vi "Latest.vi"(8 "error in (no error)":errorcluster, 10 "Migrations Folder":path, 11 "SQLite Connection in":refnum<class "Connection.lvclass">) -> (0 "error out":errorcluster, 3 "SQLite Connection out":refnum<class "Connection.lvclass">)   [LabVIEW 2024, in "DBMigrations.lvlib"]
doc: "Update database to latest version."
uses:
  DBMigrations.lvlib
  <vilib>/drjdpowell/SQLite Library/SQL Connection/Connection.lvclass
  4642a8a4-5c78-40db-aa34-a8ecced09657.vi
  <vilib>/drjdpowell/SQLite Library/SQL Connection/Execute SQL (Single Integer).vi
  <vilib>/Comparison/Less/Less Functor/Less Functor.lvclass
  <vilib>/drjdpowell/SQLite Library/SQLite.lvlib
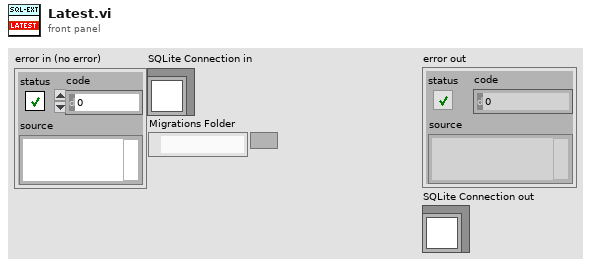
[diagram p1: front panel]
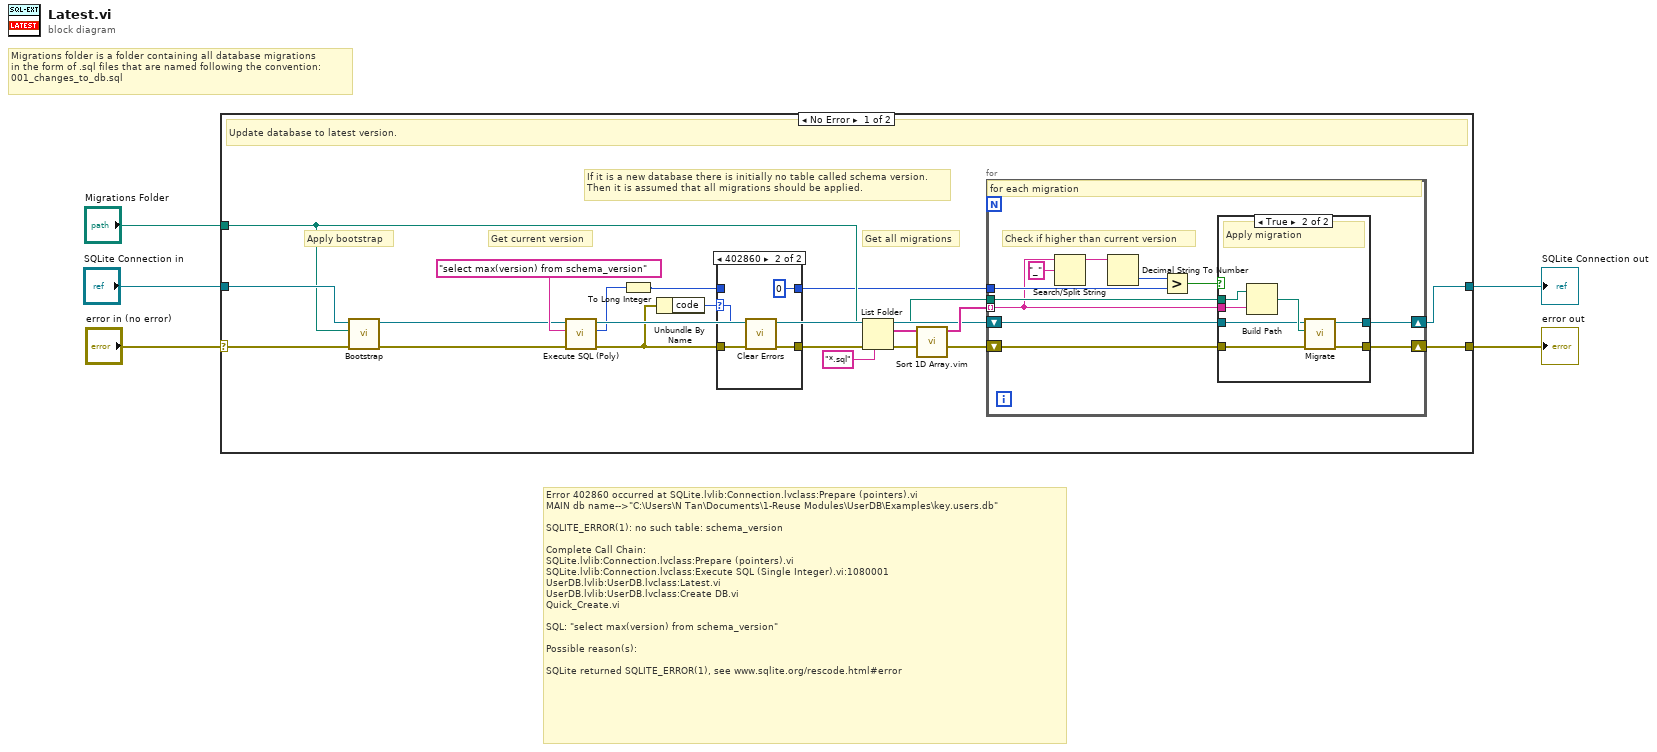
[diagram p0: block diagram]
diagram:
  # "Error 402860 occurred at SQLite.lvlib:Connection.lvclass:Prepare (pointers).vi\nMAIN db name-->\"C:\\Users\\N Tan\\Documents\\1-Reuse Modules\\UserDB\\Examples\\key.users.db\"\n\nSQLITE_ERROR(1): no such table: schema_version\n\nComplete Call Chain:\nSQLite.lvlib:Connection.lvclass:Prepare (pointers).vi\nSQLite.lvlib:Connection.lvclass:Execute SQL (Single Integer).vi:1080001\nUserDB.lvlib:UserDB.lvclass:Latest.vi\nUserDB.lvlib:UserDB.lvclass:Create DB.vi\nQuick_Create.vi\n\nSQL: \"select max(version) from schema_version\"\n\nPossible reason(s):\n\nSQLite returned SQLITE_ERROR(1), see www.sqlite.org/rescode.html#error"
  # "Migrations folder is a folder containing all database migrations\nin the form of .sql files that are named following the convention:\n001_changes_to_db.sql"
  n1 = case shown="No Error" "error in (no error)" {
    selector: "error in (no error)" -> [w15 w53]
    tunnel: [w21 w53] -> w5
    tunnel: "SQLite Connection in" -> [w14 w52]
    tunnel: [w18 w52] -> w2
    tunnel: "Migrations Folder" -> [w13 _]
    frame No Error {
      # "If it is a new database there is initially no table called schema version.\nThen it is assumed that all migrations should be applied."
      # "Get current version"
      # "Apply bootstrap"
      # "Get all migrations"
      # "Update database to latest version."
      n2 = call "Bootstrap.vi"("error in (no error)"=w15, "Migrations Folder"=w13, "SQLite Connection in"=w14) -> ("error out"=w12:errorcluster, "SQLite Connection out"=w11:refnum<class "Connection.lvclass">)  [unwired: 7 in]
      n3 = call-poly <vilib>:"Execute SQL (Poly).vi"("error in (no error)"=w12, "SQL"="select max(version) from schema_version", "SQLite Connection in"=w11) -> ("error out"=w9:errorcluster, "Result"=w16:i64, "SQLite Connection"=w20:refnum<class "Connection.lvclass">)  [unwired: 6 in]
      n4 = To Long Integer(number=w16) -> (32bit integer=w8:i32)
      n5 = Unbundle By Name(w9) -> ("code"=w10:i32)
      n6 = case shown="402860" w10 {
        selector: w10 -> [_ w28]
        tunnel: w9 -> [w27 w30]
        tunnel: [w27 w29] -> w7
        tunnel: w8 -> [w26 _]
        tunnel: [w26 0] -> w6
        frame 0, Default {
        }
        frame 402860 {
          n7 = call <vilib>:"Clear Errors.vi"("error in (no error)"=w30, "specific error code to clear (0: all)"=w28) -> ("error out"=w29:errorcluster)  [unwired: 4 in, 1 out]
        }
      }
      n8 = List Folder(path=w13, pattern="*.sql", error in=w7) -> (path out=w19:path, filenames=w24:string[], error out=w22:errorcluster)  [unwired: 1 in, 1 out]
      n9 = call "Sort 1D Array.vim"("unsorted array"=w24) -> ("sorted array"=w23:string[])  [unwired: 10 in]
      n10 = for {
        tunnel: w19 -> [w35]
        tunnel: w23 -> [w34] mode=indexing
        tunnel: w6 -> [w39]
        shift-right: [w37] -> w21
        shift-left: w22 -> [w38]
        shift-right: [w33] -> w18
        shift-left: w20 -> [w32]
        # "Check if higher than current version"
        # "for each migration"
        n11 = Search/Split String(string=w34, search string/char (-)="_" ("search string")) -> (substring before match=w41:string)  [unwired: 1 in, 2 out]
        n12 = Decimal String To Number(string=w41) -> (number=w40:i32)  [unwired: 2 in, 1 out]
        n13 = Greater?(x=w40, y=w39) -> (0:w36:bool)
        n14 = case shown="True" w36 {
          tunnel: w38 -> [w44 w51]
          tunnel: [w44 w50] -> w37
          tunnel: w35 -> [_ w49]
          tunnel: w34 -> [_ w47]
          tunnel: [w43 w46] -> w33
          tunnel: w32 -> [w43 w45]
          frame False {
            # "Skip"
          }
          frame True {
            # "Apply migration"
            n15 = Build Path(base path=w49, name or relative path=w47) -> (appended path=w48:path)
            n16 = call "Migrate.vi"("error in (no error)"=w51, "Migration File Path"=w48, "SQLite Connection in"=w45) -> ("error out"=w50:errorcluster, "SQLite Connection out"=w46:refnum<class "Connection.lvclass">)  [unwired: 7 in]
          }
        }
      }
    }
    frame Error {
    }
  }
  "error out" <- w5
  "SQLite Connection out" <- w2
